vi "VIH - CHM Project - HHP Support - Open.vi"(8 "error in":errorcluster, 10 "must exist (F)":bool, 11 "Config File":path) -> (0 "error out":errorcluster, 3 "queue out":T1)   [LabVIEW 2014]
doc: "::: VI Helpeks :::\nCopyright (c) 2000-2026 Konstantin Shifershteyn. All rights reserved."
uses:
  VIH - CHM Project - HHP Support - Queue Refnum.ctl
  VIH - CHM Project - HHP Support - Config Data Cluster.ctl
panel:
  # "VI Helpeks\nCopyright (c) 2012-2026 Konstantin Shifershteyn"
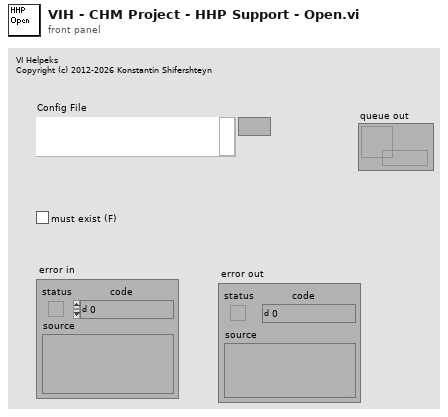
[diagram p1: front panel]
types:
  T1 = typedef "VIH - CHM Project - HHP Support - Queue Refnum.ctl" = refnum<queue>
  T2 = typedef "VIH - CHM Project - HHP Support - Config Data Cluster.ctl" = cluster{"Fille path":path, "sections":cluster{"Sec name":string, "key-values":string[][]}[]}
  T3 = cluster{"Sec name":string, "key-values":string[][]}[]
  T4 = cluster{"Sec name":string, "key-values":string[][]}
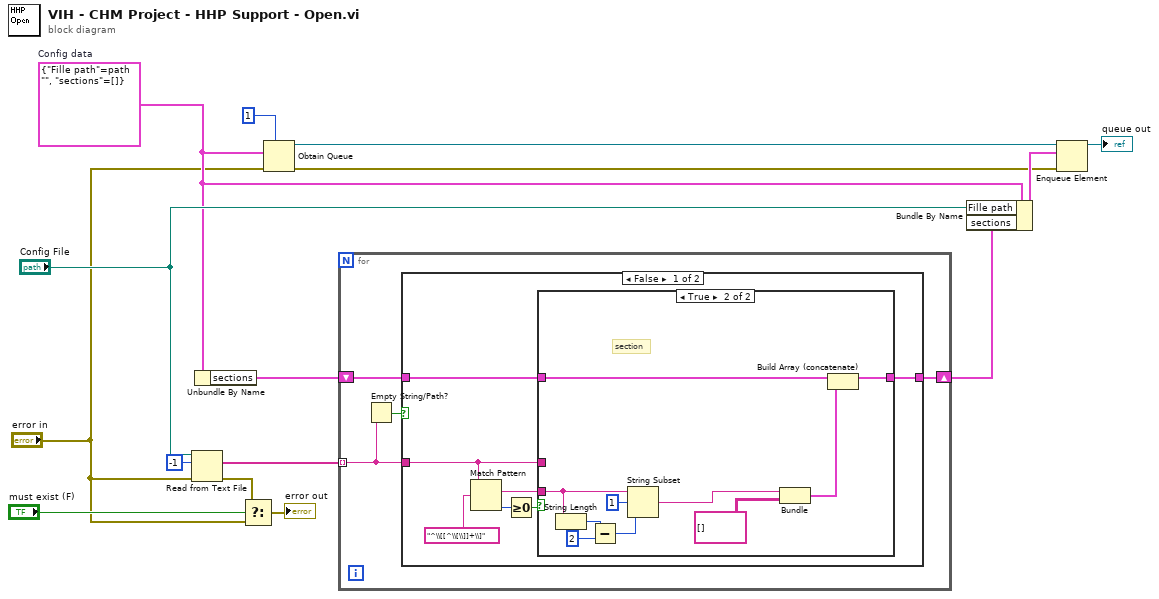
[diagram p0: block diagram]
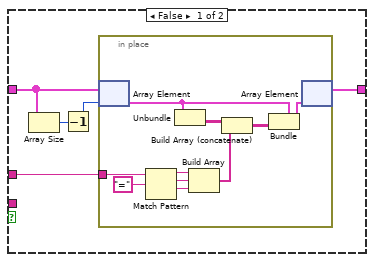
[diagram p2: hidden frame]
diagram:
  w10 = T2 {"Fille path"=path "", "sections"=[]}  # Config data
  n1 = Read from Text File(file (use dialog)="Config File", count=-1 ("count (1)"), error in="error in") -> (text=w8:string[], error out=w6:errorcluster)  [unwired: 1 in, 2 out]
  n2 = Unbundle By Name(w10) -> ("sections"=w9:T3)
  n3 = Select(t=w6, s="must exist (F)", f="error in") -> (s? t:f=→"error out":errorcluster)
  n4 = Obtain Queue(max queue size (-1, unlimited)=1, element data type=w10, error in (no error)="error in") -> (queue out=w14:refnum<queue>, error out=w7:errorcluster)  [unwired: 2 in, 1 out]
  n5 = for {
    tunnel: w8 -> [w16] mode=indexing
    shift-right: [w19] -> w2
    shift-left: w9 -> [w18]
    n6 = Empty String/Path?(string/path=w16) -> (empty?=w17:bool)
    n7 = case shown="False" w17 {
      tunnel: [w23 w52] -> w19
      tunnel: w18 -> [w22 w52]
      tunnel: w16 -> [w20 _]
      frame False {
        n8 = Match Pattern(string=w20, regular expression="^\\[[^\\[\\]]+\\]") -> (match substring=w21:string, offset past match=w25:i32)  [unwired: 1 in, 2 out]
        n9 = Greater Or Equal To 0?(x=w25) -> (x >= 0?=w24:bool)
        n10 = case shown="True" w24 {
          tunnel: [w27 w50] -> w23
          tunnel: w22 -> [w30 w51]
          tunnel: w21 -> [_ w45]
          tunnel: w20 -> [w28 _]
          frame False {
            n11 = Array Size(array=w30) -> (size(s)=w31:i32)
            n12 = Decrement(x=w31) -> (x-1=w29:i32)
            n13 = in-place {
              in-place-border: w28 -> [w37]
              n14 = in-place-array #1(w30, w29) -> (w40:T4)
              n15 = Match Pattern(string=w37, regular expression="=") -> (before substring=w35:string, match substring=w33:string, after substring=w32:string)  [unwired: 1 in, 1 out]
              n16 = Unbundle(w40) -> ("key-values"=w41:string[][])  [unwired: 1 out]
              n17 = Build Array(w35, w33, w32) -> (w34:string[])
              n18 = Build Array (concatenate)(w41, w34) -> (w39:string[][])
              n19 = Bundle(cluster=w40, "key-values"=w39) -> (w38:T4)  [unwired: 1 in]
              n20 = in-place-array #1(w38) -> (w27:T3)  [unwired: 1 out]
            }
          }
          frame True {
            # "section"
            n21 = String Length(string=w45) -> (length=w44:i32)
            n22 = Subtract(x=w44, y=2) -> (x-y=w42:i32)
            n23 = String Subset(string=w45, offset (0)=1, length (rest)=w42) -> (substring=w47:string)
            n24 = Bundle(w47, "keys"=string[][] []) -> (w48:cluster{string, "keys":string[][]})  [unwired: 1 in]
            n25 = Build Array (concatenate)(w51, w48) -> (w50:cluster{"Sec name":string, "keys":string[][]}[])
          }
        }
      }
      frame True {
      }
    }
  }
  n26 = Bundle By Name(cluster=w10, "Fille path"="Config File", "sections"=w2) -> (w13:T2)
  n27 = Enqueue Element(queue=w14, element=w13, error in (no error)=w7) -> (queue out=→"queue out":refnum<queue>)  [unwired: 1 in, 2 out]
